vi "ASD Peak-Pick Threshold VI.vi"(8 "D thred std n":dbl=5.0 format="%#_13g", 9 "U thred std n":dbl=5.0 format="%#_13g", 11 "standard deviation (pA)":dbl caption="STD (pA)" format="%0.4f") -> (0 "D thred (pA)":dbl, 1 "U thred (pA)":dbl, 2 "D thred (nA)":dbl, 3 "U thred (nA)":dbl)   [LabVIEW 2018]
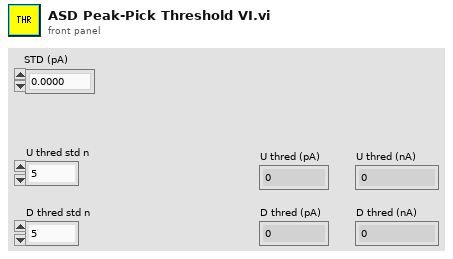
[diagram p1: front panel]
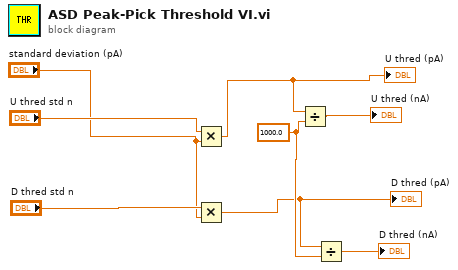
[diagram p0: block diagram]
diagram:
  w5 = 1000.0 ("x")
  n1 = Multiply(x="U thred std n", y="standard deviation (pA)") -> (x*y=w4:dbl)
  "U thred (pA)" <- w4
  n2 = Multiply(x="D thred std n", y="standard deviation (pA)") -> (x*y=w2:dbl)
  "D thred (pA)" <- w2
  n3 = Divide(x=w4, y=w5) -> (x/y=→"U thred (nA)":dbl)
  n4 = Divide(x=w2, y=w5) -> (x/y=→"D thred (nA)":dbl)
